vi "formula node using graph.vi"() -> ()   [LabVIEW 2021]
panel:
  out "Waveform Chart":dbl(graph)
  out "Numeric 2":dbl
  in  "Numeric":dbl
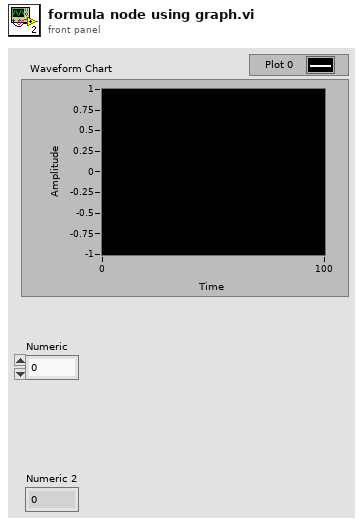
[diagram p1: front panel]
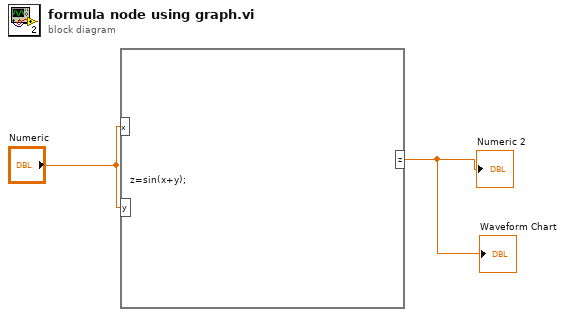
[diagram p0: block diagram]
diagram:
  n1 = formula code="z=sin(x+y);"("x"="Numeric", "y"="Numeric") -> ("z"=→"Numeric 2" →"Waveform Chart":dbl)
